vi "Pressed.vi"   [LabVIEW 2016]
uses:
  <vilib>/NXT/Block Support/NXT_InputPort.ctl
  <vilib>/NXT/Block Support/NXT_OutputPort.ctl
  <vilib>/NXT/Subs/MotorOutput.ctl
  <vilib>/NXT/Dual Mode Library/Sensors/EV3_Color_Color.vi
  <vilib>/NXT/NXTIO Xnodes/NXTIONodeSubVIs/NXTMoveMotors.vi
  <vilib>/NXT/NXTIO Xnodes/NXTIONodeSubVIs/NXTStopMotors.vi
  <vilib>/NXT/Dual Mode Library/Motors/ResetMotor.vi
  <vilib>/NXT/Dual Mode Library/Motors/Rotation.vi
  <vilib>/NXT/Dual Mode Library/Display/drawText_Center.vi
  <vilib>/NXT/Dual Mode Library/Waits/Wait_Num.vi
  <vilib>/NXT/Dual Mode Library/Display/drawNumber.vi
  <vilib>/NXT/NXTIO Xnodes/AddressXNode/NXTIOAddress.xnode
  PMR_081.lvrbt
  <vilib>/NXT/Subs/LVHSConnector.ctl
  <vilib>/NXT/NXTIO Xnodes/NXTIOXNode/NXTIO.xnode
  <vilib>/NXT/LegoClasses/BrickReference/BrickReference.lvclass
types:
  T1 = typedef "NXT_InputPort.ctl" = u32
  T2 = typedef "ColorSensorColors.ctl" = enum16{"No Color", "Black", "Blue", "Green", "Yellow", "Red", "White", "Brown"}
  T3 = typedef "NXT_OutputPort.ctl" = u8
  T4 = typedef "MotorOutput.ctl" = u8
  T5 = typedef "LVHSConnector.ctl" = refnum<class "BrickReference.lvclass">
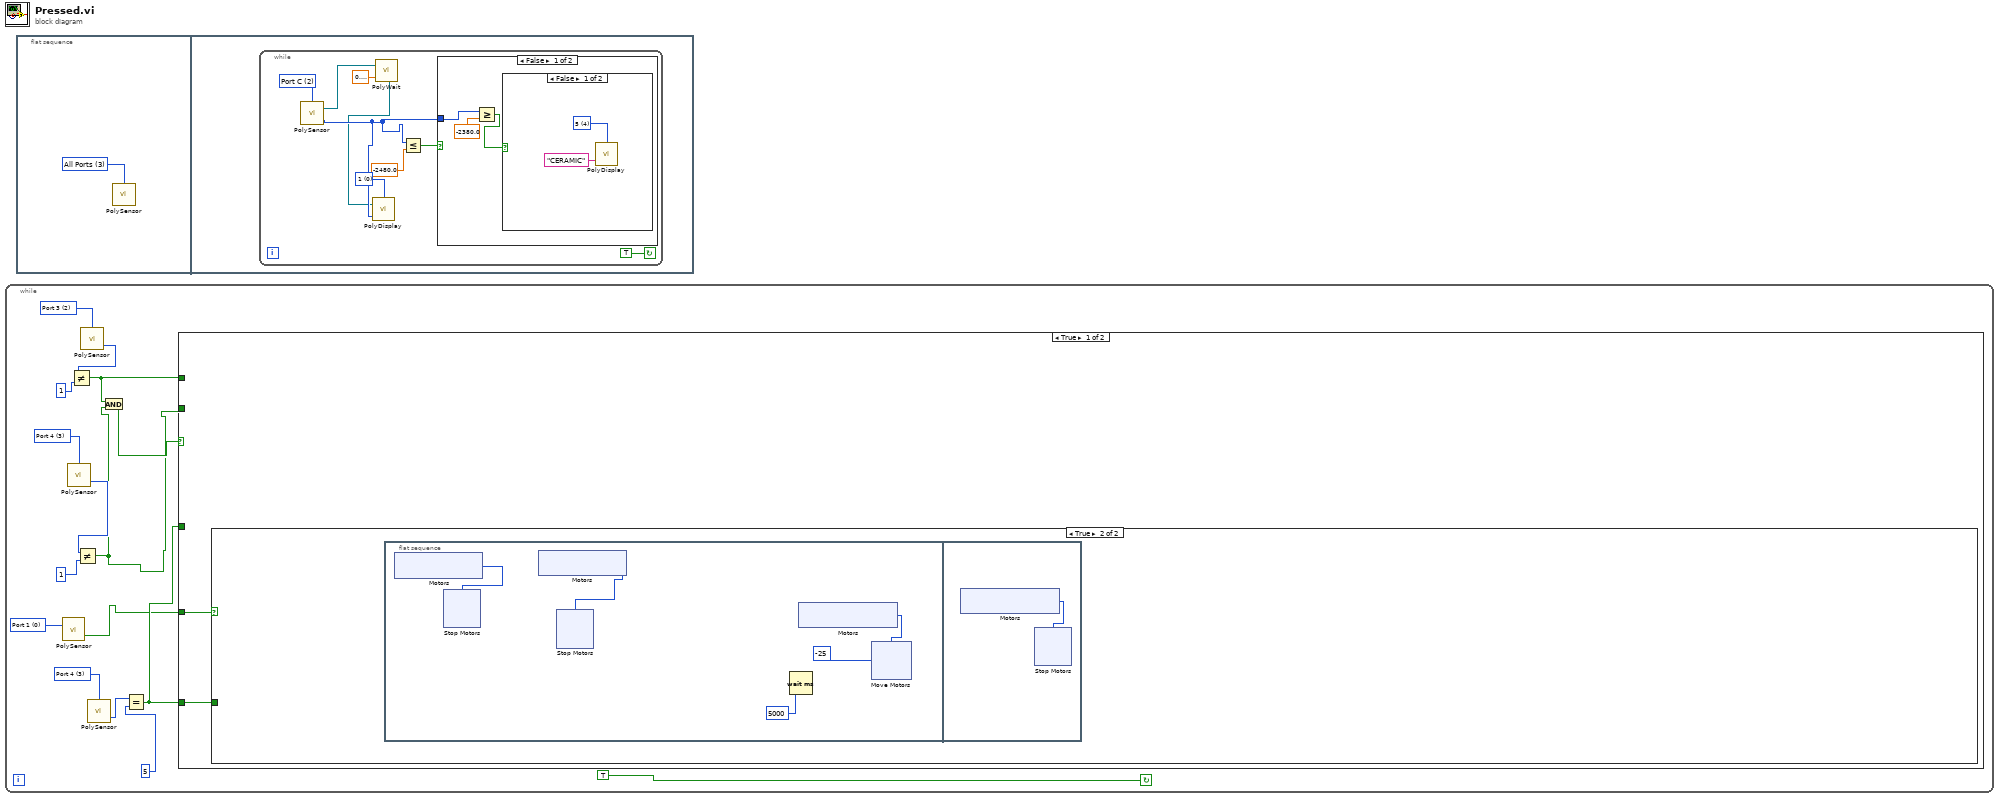
[diagram p0: block diagram]
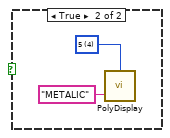
[diagram p2: hidden frame]
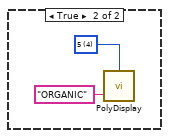
[diagram p3: hidden frame]
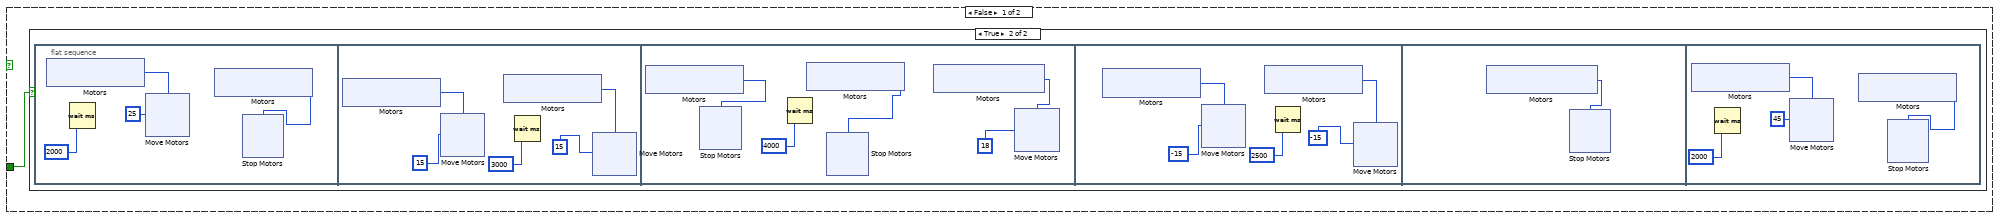
[diagram p4: hidden frame]
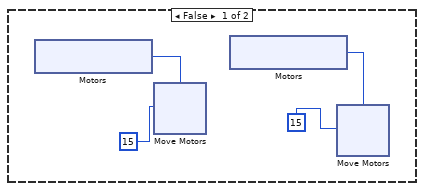
[diagram p5: hidden frame]
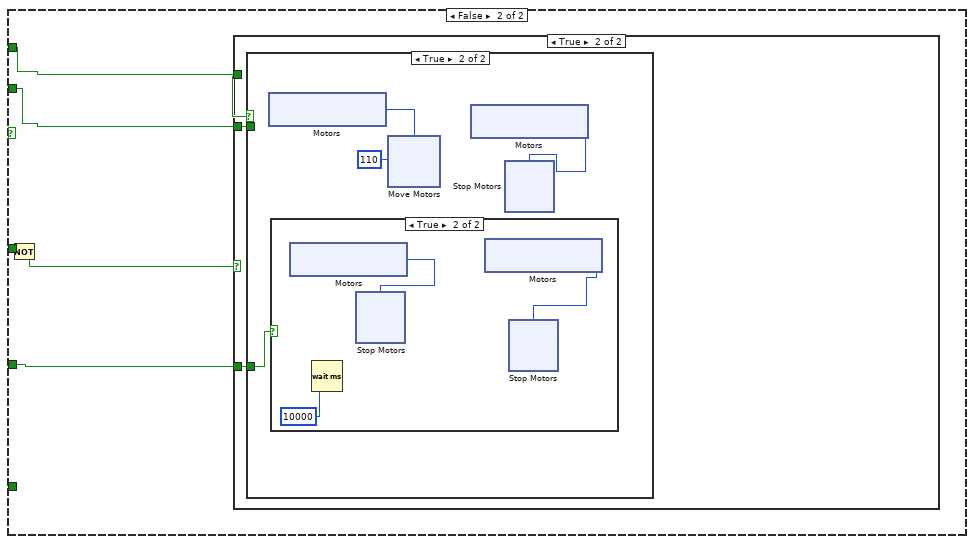
[diagram p6: hidden frame]
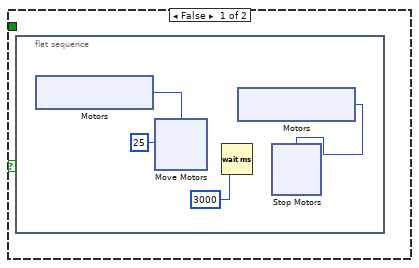
[diagram p7: hidden frame]
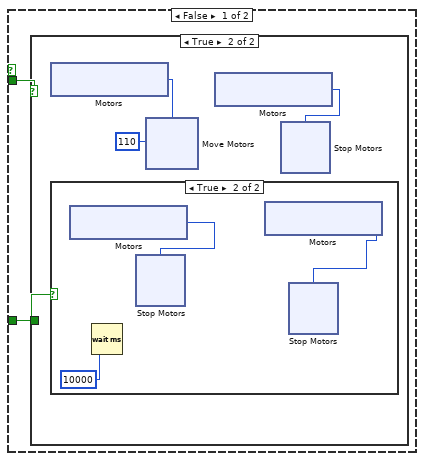
[diagram p8: hidden frame]
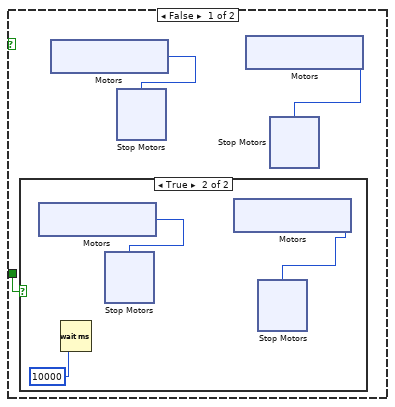
[diagram p9: hidden frame]
diagram:
  n1 = while {
    stop <- TRUE continue-if-true
    w5 = T1 3 items=["Port 1", "Port 2", "Port 3", "Port 4"] ("Port (Port 1)")
    w6 = T1 0 items=["Port 1", "Port 2", "Port 3", "Port 4"] ("Port (Port 4)")
    w15 = T1 3 items=["Port 1", "Port 2", "Port 3", "Port 4"] ("Port (Port 1)")
    w16 = T1 2 items=["Port 1", "Port 2", "Port 3", "Port 4"] ("Port (Port 1)")
    n2 = call-poly <vilib>:"PolySensor.vi"("Port (Port 1)"=w6) -> ("Yes / No"=w1:bool)  [unwired: 2 in, 1 out]
    n3 = call-poly <vilib>:"PolySensor.vi"("Port (Port 1)"=w15) -> ("Detected Color"=w11:T2)  [unwired: 2 in, 1 out]
    n4 = Not Equal?(x=w11, y=1) -> (x != y?=w7:bool)
    n5 = call-poly <vilib>:"PolySensor.vi"("Port (Port 1)"=w16) -> ("Detected Color"=w13:T2)  [unwired: 2 in, 1 out]
    n6 = Not Equal?(x=w13, y=1) -> (x != y?=w9:bool)
    n7 = call-poly <vilib>:"PolySensor.vi"("Port (Port 1)"=w5) -> ("Detected Color"=w4:T2)  [unwired: 2 in, 1 out]
    n8 = And(x=w9, y=w7) -> (x .and. y?=w8:bool)
    n9 = Equal?(x=w4, y=5) -> (x = y?=w2:bool)
    n10 = case shown="True" w8 {
      tunnel: w9 -> [_ w186]
      tunnel: w7 -> [_ w185]
      tunnel: w1 -> [w18 w184]
      tunnel: w2 -> [w17 _]
      tunnel: w2 -> [_ w183]
      frame True {
        n11 = case shown="True" w18 {
          tunnel: w17 -> [w19 _]
          frame False {
            n12 = case shown="True" w19 {
              frame False {
                n13 = xnode "Motors"() -> ("Motor"=w22:T3)
                n14 = xnode "Move Motors"("Power/Speed 1"=i8 15, "Motors"=w22) -> ()  [unwired: 1 in, 1 out]
                n15 = xnode "Motors"() -> ("Motor"=w23:T3)
                n16 = xnode "Move Motors"("Power/Speed 1"=i8 15, "Motors"=w23) -> ()  [unwired: 1 in, 1 out]
              }
              frame True {
                n17 = flat-sequence {
                  frame #0 {
                    n18 = xnode "Motors"() -> ("Motor"=w42:T3)
                    n19 = Wait (ms)(milliseconds to wait=2000) -> ()  [unwired: 1 out]
                    n20 = xnode "Move Motors"("Power/Speed 1"=i8 25, "Motors"=w42) -> ()  [unwired: 1 in, 1 out]
                    n21 = xnode "Motors"() -> ("Motor"=w41:T3)
                    n22 = xnode "Stop Motors"("Motors"=w41) -> ()  [unwired: 1 in, 1 out]
                  }
                  frame #1 {
                    n23 = xnode "Motors"() -> ("Motor"=w61:T3)
                    n24 = xnode "Move Motors"("Power/Speed 1"=i8 15, "Motors"=w61) -> ()  [unwired: 1 in, 1 out]
                    n25 = xnode "Motors"() -> ("Motor"=w62:T3)
                    n26 = Wait (ms)(milliseconds to wait=3000) -> ()  [unwired: 1 out]
                    n27 = xnode "Move Motors"("Power/Speed 1"=i8 15, "Motors"=w62) -> ()  [unwired: 1 in, 1 out]
                  }
                  frame #2 {
                    n28 = xnode "Motors"() -> ("Motor"=w82:T3)
                    n29 = xnode "Stop Motors"("Motors"=w82) -> ()  [unwired: 1 in, 1 out]
                    n30 = Wait (ms)(milliseconds to wait=4000) -> ()  [unwired: 1 out]
                    n31 = xnode "Motors"() -> ("Motor"=w81:T3)
                    n32 = xnode "Stop Motors"("Motors"=w81) -> ()  [unwired: 1 in, 1 out]
                    n33 = xnode "Motors"() -> ("Motor"=w79:T3)
                    n34 = xnode "Move Motors"("Power/Speed 1"=18, "Motors"=w79) -> ()  [unwired: 1 in, 1 out]
                  }
                  frame #3 {
                    n35 = xnode "Motors"() -> ("Motor"=w107:T3)
                    n36 = xnode "Move Motors"("Power/Speed 1"=i8 -15, "Motors"=w107) -> ()  [unwired: 1 in, 1 out]
                    n37 = xnode "Motors"() -> ("Motor"=w108:T3)
                    n38 = Wait (ms)(milliseconds to wait=2500) -> ()  [unwired: 1 out]
                    n39 = xnode "Move Motors"("Power/Speed 1"=i8 -15, "Motors"=w108) -> ()  [unwired: 1 in, 1 out]
                  }
                  frame #4 {
                    n40 = xnode "Motors"() -> ("Motor"=w125:T3)
                    n41 = xnode "Stop Motors"("Motors"=w125) -> ()  [unwired: 1 in, 1 out]
                  }
                  frame #5 {
                    n42 = xnode "Motors"() -> ("Motor"=w133:T3)
                    n43 = Wait (ms)(milliseconds to wait=2000) -> ()  [unwired: 1 out]
                    n44 = xnode "Move Motors"("Power/Speed 1"=i8 45, "Motors"=w133) -> ()  [unwired: 1 in, 1 out]
                    n45 = xnode "Motors"() -> ("Motor"=w134:T3)
                    n46 = xnode "Stop Motors"("Motors"=w134) -> ()  [unwired: 1 in, 1 out]
                  }
                }
              }
            }
          }
          frame True {
            n47 = flat-sequence {
              frame #0 {
                n48 = xnode "Motors"() -> ("Motor"=w154:T3)
                n49 = xnode "Stop Motors"("Motors"=w154) -> ()  [unwired: 1 in, 1 out]
                n50 = xnode "Motors"() -> ("Motor"=w153:T3)
                n51 = xnode "Stop Motors"("Motors"=w153) -> ()  [unwired: 1 in, 1 out]
                n52 = Wait (ms)(milliseconds to wait=5000) -> ()  [unwired: 1 out]
                n53 = xnode "Motors"() -> ("Motor"=w150:T3)
                n54 = xnode "Move Motors"("Power/Speed 1"=-25, "Motors"=w150) -> ()  [unwired: 1 in, 1 out]
              }
              frame #1 {
                n55 = xnode "Motors"() -> ("Motor"=w175:T3)
                n56 = xnode "Stop Motors"("Motors"=w175) -> ()  [unwired: 1 in, 1 out]
              }
            }
          }
        }
      }
      frame False {
        n57 = Not(x=w183) -> (.not. x?=w182:bool)
        n58 = case shown="True" w182 {
          tunnel: w186 -> [_ w207]
          tunnel: w185 -> [_ w206]
          tunnel: w184 -> [_ w205]
          frame False {
            n59 = flat-sequence {
              frame #0 {
                n60 = xnode "Motors"() -> ("Motor"=w189:T3)
                n61 = xnode "Move Motors"("Power/Speed 1"=i8 25, "Motors"=w189) -> ()  [unwired: 1 in, 1 out]
                n62 = Wait (ms)(milliseconds to wait=3000) -> ()  [unwired: 1 out]
                n63 = xnode "Motors"() -> ("Motor"=w188:T3)
                n64 = xnode "Stop Motors"("Motors"=w188) -> ()  [unwired: 1 in, 1 out]
              }
            }
          }
          frame True {
            n65 = case shown="True" w207 {
              tunnel: w206 -> [w209 _]
              tunnel: w205 -> [w208 w273]
              frame False {
                n66 = case shown="True" w209 {
                  tunnel: w208 -> [w210 w240]
                  frame False {
                    n67 = case shown="True" w210 {
                      frame False {
                      }
                      frame True {
                        n68 = xnode "Motors"() -> ("Motor"=w214:T3)
                        n69 = Wait (ms)(milliseconds to wait=10000) -> ()  [unwired: 1 out]
                        n70 = xnode "Stop Motors"("Motors"=w214) -> ()  [unwired: 1 in, 1 out]
                        n71 = xnode "Motors"() -> ("Motor"=w213:T3)
                        n72 = xnode "Stop Motors"("Motors"=w213) -> ()  [unwired: 1 in, 1 out]
                      }
                    }
                    n73 = xnode "Motors"() -> ("Motor"=w211:T3)
                    n74 = xnode "Stop Motors"("Motors"=w211) -> ()  [unwired: 1 in, 1 out]
                    n75 = xnode "Motors"() -> ("Motor"=w212:T3)
                    n76 = xnode "Stop Motors"("Motors"=w212) -> ()  [unwired: 1 in, 1 out]
                  }
                  frame True {
                    n77 = xnode "Motors"() -> ("Motor"=w242:T3)
                    n78 = case shown="True" w240 {
                      frame False {
                      }
                      frame True {
                        n79 = xnode "Motors"() -> ("Motor"=w245:T3)
                        n80 = Wait (ms)(milliseconds to wait=10000) -> ()  [unwired: 1 out]
                        n81 = xnode "Stop Motors"("Motors"=w245) -> ()  [unwired: 1 in, 1 out]
                        n82 = xnode "Motors"() -> ("Motor"=w244:T3)
                        n83 = xnode "Stop Motors"("Motors"=w244) -> ()  [unwired: 1 in, 1 out]
                      }
                    }
                    n84 = xnode "Move Motors"("Power/Speed 1"=i8 110, "Motors"=w242) -> ()  [unwired: 1 in, 1 out]
                    n85 = xnode "Motors"() -> ("Motor"=w243:T3)
                    n86 = xnode "Stop Motors"("Motors"=w243) -> ()  [unwired: 1 in, 1 out]
                  }
                }
              }
              frame True {
                n87 = xnode "Motors"() -> ("Motor"=w275:T3)
                n88 = case shown="True" w273 {
                  frame False {
                  }
                  frame True {
                    n89 = xnode "Motors"() -> ("Motor"=w283:T3)
                    n90 = Wait (ms)(milliseconds to wait=10000) -> ()  [unwired: 1 out]
                    n91 = xnode "Stop Motors"("Motors"=w283) -> ()  [unwired: 1 in, 1 out]
                    n92 = xnode "Motors"() -> ("Motor"=w282:T3)
                    n93 = xnode "Stop Motors"("Motors"=w282) -> ()  [unwired: 1 in, 1 out]
                  }
                }
                n94 = xnode "Move Motors"("Power/Speed 1"=i8 110, "Motors"=w275) -> ()  [unwired: 1 in, 1 out]
                n95 = xnode "Motors"() -> ("Motor"=w274:T3)
                n96 = xnode "Stop Motors"("Motors"=w274) -> ()  [unwired: 1 in, 1 out]
              }
            }
          }
        }
      }
    }
  }
  n97 = flat-sequence {
    frame #0 {
      w306 = T4 3 items=["Port A"=0, "Port B"=1, "Port C"=2, "Ports A & B"=4, "Ports A & C"=5, "Ports B & C"=6, "All Ports"=3] ("Port (All Ports)")
      n98 = call-poly <vilib>:"PolySensor.vi"("Port (All Ports)"=w306) -> ()  [unwired: 3 in, 1 out]
    }
    frame #1 {
      n99 = while {
        stop <- TRUE continue-if-true
        w311 = i16 0 items=["1", "2", "3", "4", "5", "6", "7", "8", "9", "10", "11", "12"] ("Line")
        w312 = T3 2 items=["Port A", "Port B", "Port C", "Port D"] ("Port (Port A)")
        n100 = call-poly <vilib>:"PolySensor.vi"("Port (Port A)"=w312) -> ("Angle of Rotation"=w310:i32, "NXT/EV3"=w309:T5)  [unwired: 2 in]
        n101 = call-poly <vilib>:"PolyWait.vi"("Time (1 sec)"=sgl 0.3, "NXT/EV3"=w309) -> ("NXT/EV3"=w308:T5)  [unwired: 2 in]
        n102 = call-poly <vilib>:"PolyDisplay.vi"("number"=w310, "NXT/EV3"=w308, "Line"=w311) -> ()  [unwired: 1 in, 1 out]
        n103 = Less Or Equal?(x=w310, y=sgl -2480.0) -> (x <= y?=w314:bool)
        n104 = case shown="False" w314 {
          tunnel: w310 -> [w317 _]
          frame False {
            n105 = Greater Or Equal?(x=w317, y=sgl -2380.0) -> (x >= y?=w316:bool)
            n106 = case shown="False" w316 {
              frame False {
                w319 = i16 4 items=["1", "2", "3", "4", "5", "6", "7", "8", "9", "10", "11", "12"] ("Line")
                n107 = call-poly <vilib>:"PolyDisplay.vi"("Text"="CERAMIC", "Line"=w319) -> ()  [unwired: 2 in, 1 out]
              }
              frame True {
                w321 = i16 4 items=["1", "2", "3", "4", "5", "6", "7", "8", "9", "10", "11", "12"] ("Line")
                n108 = call-poly <vilib>:"PolyDisplay.vi"("Text"="METALIC", "Line"=w321) -> ()  [unwired: 2 in, 1 out]
              }
            }
          }
          frame True {
            w323 = i16 4 items=["1", "2", "3", "4", "5", "6", "7", "8", "9", "10", "11", "12"] ("Line")
            n109 = call-poly <vilib>:"PolyDisplay.vi"("Text"="ORGANIC", "Line"=w323) -> ()  [unwired: 2 in, 1 out]
          }
        }
      }
    }
  }
